vi "New.vi"(8 "error in (no error)":errorcluster, 11 "ChannelMap":map{string, T1}(c390)) -> (0 "error out":errorcluster, 3 "StokePlotHandle out":refnum<class "BjusticePlotHandle.lvclass">)   [LabVIEW 2021, in "BjusticePlotHandle.lvclass"]
uses:
  BjusticePlotHandle.lvclass
  <userlib>/bjustice/Ring Buffer for Time Series Data Strict Accessor/SubVIs/RingBufferHandle.ctl
  <userlib>/bjustice/Ring Buffer for Time Series Data/SubVIs/DVR data.ctl
  <userlib>/bjustice/Ring Buffer for Time Series Data Strict Accessor/SubVIs/DataType.ctl
  <userlib>/bjustice/Ring Buffer for Time Series Data Strict Accessor/SubVIs/Endianess.ctl
  BjusticePlotHandle.lvclass/BjusticePlotHandle.ctl
  <userlib>/bjustice/Ring Buffer for Time Series Data/Ring Buffer Time Series Data.lvlib
  <userlib>/bjustice/Ring Buffer for Time Series Data Strict Accessor/Ring Buffer Strict Accessor.lvlib
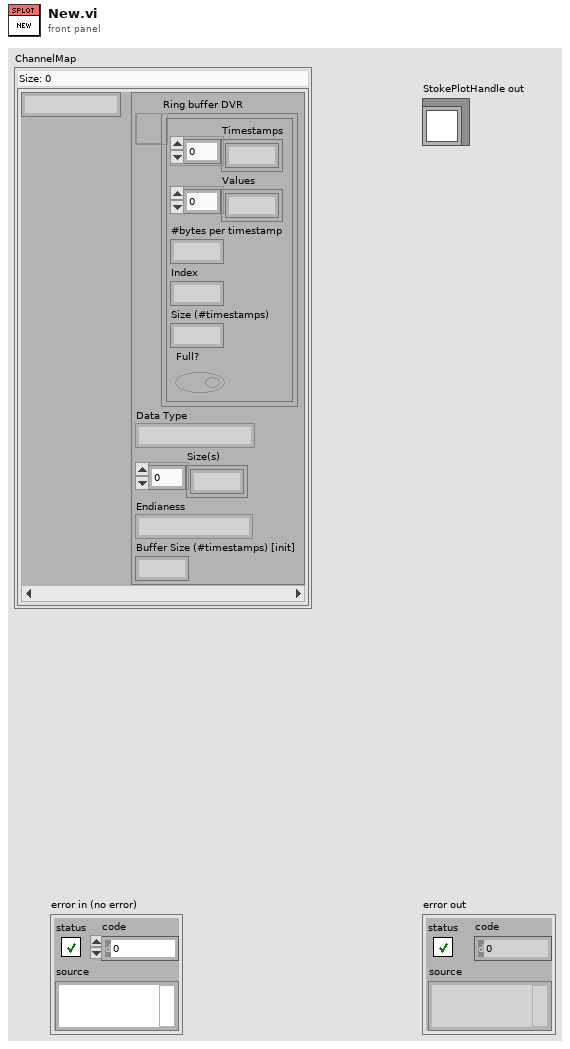
[diagram p1: front panel]
types:
  T1 = typedef "Ring Buffer Strict Accessor.lvlib/RingBufferHandle.ctl" = cluster{"Ring buffer DVR":refnum<data-value>, "Data Type":T2, "Size(s)":i32[], "Endianess":T3, "Buffer Size (#timestamps) [init]":i32}
  T2 = typedef "Ring Buffer Strict Accessor.lvlib/DataType.ctl" = enum16{"uint8", "uint16", "uint32", "uint64", "int8", "int16", "int32", "int64", "float", "double", "extended"}
  T3 = typedef "Ring Buffer Strict Accessor.lvlib/Endianess.ctl" = enum16{"big-endian", "little-endian"}
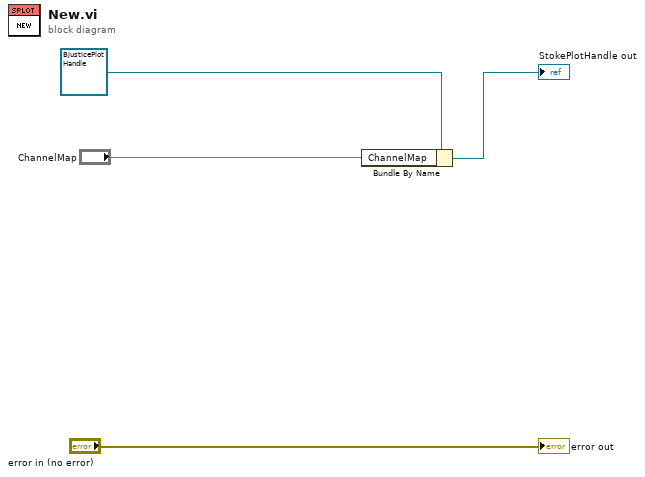
[diagram p0: block diagram]
diagram:
  n1 = Bundle By Name(cluster=refnum<class "BjusticePlotHandle.lvclass"> refnum ("StokePlotHandle out"), "ChannelMap"="ChannelMap") -> (→"StokePlotHandle out":refnum<class "BjusticePlotHandle.lvclass">)
  "error out" <- "error in (no error)"
